vi "Stop Condition - Saturation 1 (SubVI) (1).vi"(6 "Enum":enum16{"Saturation", "B-Check"}(ring), 8 "error in (no error)":errorcluster, 9 "Test RunTime":dbl, 10 "Time":dbl, 11 "Cluster in":T1 {"M Event" items=["Stop", "Running", "PID", "Up Limit", "Down Limit", "Load Limit"]; "Test Type" items=["Please Select", "Triaxial Shear", "Triaxial UU", "Shearbox", "Permeability", "Consolidation (Stepped Loading)/Swelling", "Saturation (Incremental)", "User Defined", "UCT", "Isotropic Consolidation", "Swelling Pressure", "B-Check", "Saturation (Step Increment)", "Saturation (Ramp)"]; "Data"."Test Type" items=["Please Select", "Triaxial Shear", "Triaxial UU", "Shearbox", "Permeability", "Consolidation (Stepped Loading)/Swelling", "Saturation (Incremental)", "User Defined", "UCT", "Isotropic Consolidation", "Swelling Pressure", "B-Check", "Saturation (Step Increment)", "Saturation (Ramp)"]}) -> (0 "error out":errorcluster, 3 "Cluster out":T1 {"M Event" items=["Stop", "Running", "PID", "Up Limit", "Down Limit", "Load Limit"]; "Test Type" items=["Please Select", "Triaxial Shear", "Triaxial UU", "Shearbox", "Permeability", "Consolidation (Stepped Loading)/Swelling", "Saturation (Incremental)", "User Defined", "UCT", "Isotropic Consolidation", "Swelling Pressure", "B-Check", "Saturation (Step Increment)", "Saturation (Ramp)"]; "Data"."Test Type" items=["Please Select", "Triaxial Shear", "Triaxial UU", "Shearbox", "Permeability", "Consolidation (Stepped Loading)/Swelling", "Saturation (Incremental)", "User Defined", "UCT", "Isotropic Consolidation", "Swelling Pressure", "B-Check", "Saturation (Step Increment)", "Saturation (Ramp)"]}, 4 "Delay":string, 7 "Log?":bool)   [LabVIEW 2019]
uses:
  Controls/RunTest - Data Structure.ctl
  Controls/Test Panel - Data Structure.ctl
  Controls/Station - Test Type.ctl
  <vilib>/Utility/miscctls.llb/LVRowAndColumnTypeDef.ctl
  Controls/RunTest - Calculate Data.ctl
  <vilib>/httpClient/ClientHandle.ctl
  Controls/RunTest - Start Condition.ctl
  Controls/RunTest - Stop Condition.ctl
  Controls/UDP - Event.ctl
  Controls/eFGV States.ctl
  <vilib>/httpClient/LabVIEWHTTPClient.lvlib
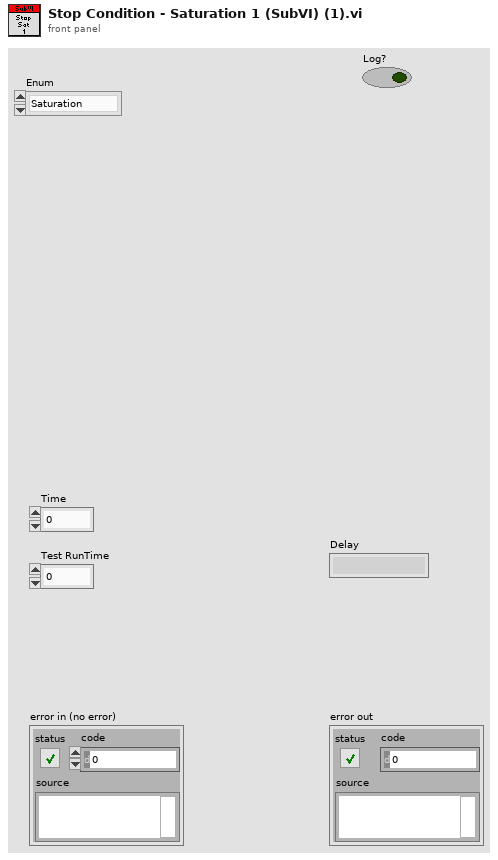
[diagram p1: front panel]
types:
  T1 = typedef "RunTest - Data Structure.ctl" = cluster{"Test Plan":string[], "PlanRow":i32, "Device Name":string[], "Timeout":i32, "Start?":bool, "Pause?":bool, "IP Address":string[], "LogRow":i32, "Logtype":u16, "Log Elapse":sgl, "Data":T2, "Stop log?":bool, "tdms":refnum<k34>, "Sensor Data":sgl[], "Start time":timestamp, "Prev Log Elapse":u32, "Plot":u16, "X-Axis":u16[], "Y-Axis":u16[], "XY":cluster{"X":dbl, "Y":dbl}[][], "End Stage?":bool, "1run":bool, "Condition":u16[], "Start Con":bool, "Log Con":bool, "Stop Con":bool, "Start Elapse":dbl, "Start Load":dbl, "Motor":i32, "StartRow":i32, "number log":i32, "Dir":bool, "Start time test":timestamp, "Auto":bool, "Check return?":bool, "Inv":cluster{"M":i32[], "Bool":bool[]}, "tdms temp":refnum<k34>, "Zero?":bool, "Plot Timer":dbl, "1st Run":bool, "TDMS Path":path, "MaxLoad":dbl, "Log Timer":sgl[], "Test Type":T3, "Log Sensor":string[], "Save?":bool, "1st Log":bool, "Y-Axis 2":u16[], "On Y-Axis 2":bool, "Decimal":u8[], "Init":cluster{"PWP TS":sgl, "Load TS":sgl, "Volume TS":sgl, "Disp TS":sgl, "CP":sgl, "Vol In":sgl, "Vol Out":sgl, "Load UCT":sgl, "Disp UCT":sgl, "PWP Sat":sgl, "CP Sat":sgl, "Volume IsoCons":sgl, "PWP IsoCons":sgl, "PWP TUU":sgl, "Load TUU":sgl, "Volume TUU":sgl, "Disp TUU":sgl, "Load Cons":sgl, "Disp Cons":sgl, "Volume Sat":sgl, "Vertical Load SB":sgl, "Vertical Disp SB":sgl, "H Disp SB":sgl, "H Load SB":sgl, "PWP BC":sgl, "CP BC":sgl, "PWP Sat Step":sgl, "CP Sat Step":sgl, "Volume Sat Step":sgl, "PWP Sat Ramp":sgl, "CP Sat Ramp":sgl, "Volume Sat Ramp":sgl}, "Calc":T5, "Device Index":i32[], "Channel Index":i32[], "http ref":T6, "fileid":string, "Step Cons":cluster{"V Stress":sgl, "H Settlement":sgl}, "RunTest":bool, "Graph Last":i32, "Init?":bool, "Datalog":bool[], "Start":T7, "Stop":T8, "Running?":bool, "StartTime":dbl, "Log Prev Time":dbl, "KeyName":string[], "Test RunTime":dbl, "Log Prev Axial":dbl, "M Event":T9[], "Last Log":bool, "popup":bool, "PreStart UU":bool, "PreStart Sat":bool, "PreStart BC":bool, "PreStart Sat Step":bool, "PreStart Sat Ramp":bool, "Prev Sat IP":string}
  T2 = typedef "Test Panel - Data Structure.ctl" = cluster{"Station":string, "Sample ID":string, "Job No":string, "Job Description":string, "Filename":string, "Test Type":T3, "Speciment No":string, "Depth":string, "Height":string, "Diameter/Length":string, "Weight":string, "Test Parameter":string, "Station[]":string[], "Edit Pos":T4, "Edit Pos Prev":T4, "Area":string, "Path":string, "sample_id":string}
  T3 = typedef "Station - Test Type.ctl" = u16
  T4 = typedef "LVRowAndColumnTypeDef.ctl" = cluster{"Row":i32, "Column":i32}
  T5 = typedef "RunTest - Calculate Data.ctl" = cluster{"TS":cluster{"Change PWP":sgl, "Change Vol":sgl, "Axial Load":sgl, "CiL":sgl, "Deviator":sgl, "Axial Strain":sgl, "MaxDeviator":sgl, "SS":sgl, "CAS":sgl}, "TUU":cluster{"Change PWP":sgl, "Axial Load":sgl, "CiL":sgl, "Deviator":sgl, "Axial Strain":sgl, "MaxDeviator":sgl}, "Sat":cluster{"B Value":sgl, "PWP Diss":sgl, "CPP":sgl, "CV":sgl}, "Per":cluster{"Change Vol In":sgl, "Change Vol Out":sgl, "Mean Vol":sgl, "Gradient Pressure":sgl, "Outlet Flow":sgl, "Inlet Flow":sgl, "I X1":sgl, "I X2":sgl, "I Y1":sgl, "I Y2":sgl, "O X1":sgl, "O X2":sgl, "O Y1":sgl, "O Y2":sgl}, "Step Cons":cluster{"V Stress":sgl, "H Settlement":sgl, "Total H Settle":sgl, "Prev Total H":sgl}, "UCT":cluster{"ALC":sgl, "H Change":sgl, "Deviator":sgl, "Axial Strain":sgl, "V Stress":sgl, "MaxDeviator":sgl}, "ISO Cons":cluster{"CPP":sgl, "PWP Diss":sgl, "CV":sgl, "VS":sgl}, "SB":cluster{"Speci LenC":sgl, "Shear Strain":sgl, "H LC":sgl, "Normal Stress":sgl, "Shear Stress":sgl, "MaxShear":sgl}, "BC":cluster{"B Value":sgl, "PWP Diss":sgl, "CPP":sgl, "CV":sgl}, "Sat Step":cluster{"B Value":sgl, "PWP Diss":sgl, "CPP":sgl, "CV":sgl}, "Sat Ramp":cluster{"B Value":sgl, "PWP Diss":sgl, "CPP":sgl, "CV":sgl}, "Prev Log":string[]}
  T6 = typedef "LabVIEWHTTPClient.lvlib/ClientHandle.ctl" = refnum<k1>
  T7 = typedef "RunTest - Start Condition.ctl" = cluster{"Cons":cluster{"VS":dbl, "Delay":bool, "No Delay":dbl}, "Sat":cluster{"CP":dbl, "BP":dbl, "StartBP":bool, "Target CP":bool, "Target BP":bool}, "Iso":cluster{"Select":dbl, "BP":dbl, "IC2":dbl, "IC3":dbl, "IC4":dbl, ". IC6":bool, "IC6":dbl, "IC6-2":dbl, "Time Cond":dbl, "Last PWP":dbl, "Target CP":bool, "Target BP":bool, "NewCP":dbl, "NewBP":dbl, "Noti CP":bool, "Noti BP":bool, "Noti PWP":bool, "PrevSatBP":dbl}, "TS":cluster{"SS":dbl, "Engage":bool, "ES":dbl, "LC":dbl, "PreStart":bool, "Trig SS":bool, "Drain":dbl, "Select":u16, "Max SS .":bool, "MaxSS":dbl}, "TUU":cluster{"SS":dbl, "Engage":bool, "ES":dbl, "LC":dbl, "PreStart":bool, "Trig SS":bool, "CP":dbl, "Delay Value":dbl, "Delay":bool, "CP PID":bool}, "UCT":cluster{"SS":dbl, "Engage":bool, "ES":dbl, "LC":dbl, "PreStart":bool, "Trig SS":bool}, "Enable?":bool, "SB":cluster{"SS":dbl, "Engage":bool, "ES":dbl, "LC":dbl, "PreStart":bool, "Trig SS":bool, "VS":dbl, "Delay Value":dbl, "Delay":bool, "VS PID":bool}, "Perm":cluster{"DP":dbl}, "BC":cluster{"CP":dbl, "Target CP":bool, "Target BP":bool, "CP Inc":dbl, "CP .Init":bool, "CP Init":dbl, "1st BC":bool}, "Sat (Step)":cluster{"Select":dbl, "CP":dbl, "BP":dbl, "EP":dbl, "StartCP":bool, "Target CP":bool, "Target BP":bool}, "Sat (Ramp)":cluster{"Select":dbl, "CP":dbl, "BP":dbl, "EP":dbl, "StartCP":bool, "Target CP":bool, "Target BP":bool, "Time Rate":u32}}
  T8 = typedef "RunTest - Stop Condition.ctl" = cluster{"Cons":cluster{"Select":i32, "Disp":dbl, "Time":dbl, "Time2":dbl, "Disp 2":dbl, "Time Cond":dbl, "Last Disp":dbl, "Swell":bool, "T50,90,100":cluster{"t50_x_min":dbl, "t50_y_value":dbl, "t90_x_min":dbl, "t90_y_value":dbl, "t100_x_min":dbl, "t100_y_value":dbl, "target_column":string, "test_type":string, "error":string}}, "Sat":cluster{"Select":i32, "PP":dbl, "Time":dbl, "VC":dbl, "Time2":dbl, "Time Cond":dbl, "Last PP":dbl, ".B":bool, "B":dbl, "Last Vc":dbl, "Time Cond 2":dbl, "Time3":dbl, "Time Cond 3":dbl, "B Achieve":bool, "PP Achieve":bool, "VC Achieve":bool, "Max Achieve":bool, "CP Check":dbl, "Skip Next":bool, "B Achieve Stage":u32, ".CP Check":bool}, "Iso":cluster{"PP":dbl, "Time":dbl, "VC":dbl, "Time2":dbl, "Time Cond":dbl, "Last Vc":dbl, ".PP":bool, "Time Cond 2":dbl, "Select":i32, "BS":cluster{"t50_x_min":dbl, "t50_y_value":dbl, "t90_x_min":dbl, "t90_y_value":dbl, "t100_x_min":dbl, "t100_y_value":dbl, "target_column":string, "test_type":string, "error":string}, "Final VC":dbl, "ASTM":cluster{"t50_x_min":dbl, "t50_y_value":dbl, "t90_x_min":dbl, "t90_y_value":dbl, "t100_x_min":dbl, "t100_y_value":dbl, "target_column":string, "test_type":string, "error":string}, "ASTM Log":cluster{"t50_x_min":dbl, "t50_y_value":dbl, "t90_x_min":dbl, "t90_y_value":dbl, "t100_x_min":dbl, "t100_y_value":dbl, "target_column":string, "test_type":string, "error":string}, "PP Achieve":bool, "VC Achieve":bool}, "TS":cluster{"Axial":dbl, ".MaxDev":bool, "MaxDev Value":dbl, "Return":bool, "Reset":bool, "Prev Time":dbl, "PostStop Run":bool, "CP Stop":bool, "BP Stop":bool, "PostStop Trig":bool, "Reset Value":dbl, "BPTrig":bool, "CPTrig":bool, "VLCTrig":bool, "CAxial":dbl, "Select":i32}, "TUU":cluster{"Axial":dbl, ".MaxDev":bool, "MaxDev Value":dbl, "Return":bool, "Reset":bool, "Prev Time":dbl, "PostStop Run":bool, "CP Stop":bool, "BP Stop":bool, "PostStop Trig":bool, "Reset Value":dbl, "BPTrig":bool, "CPTrig":bool, "VLCTrig":bool}, "UCT":cluster{"Axial":dbl, ".MaxDev":bool, "MaxDev Value":dbl, "Return":bool, "Reset":bool, "Prev Time":dbl, "PostStop Run":bool, "CP Stop":bool, "BP Stop":bool, "PostStop Trig":bool}, "Enable?":bool, "SB":cluster{"Shear":dbl, ".MaxShear":bool, "MaxShear Value":dbl, "Return":bool, "Reset":bool, "Prev Time":dbl, "PostStop Run":bool, "CP Stop":bool, "BP Stop":bool, "PostStop Trig":bool, "Reset Value":dbl, "BPTrig":bool, "CPTrig":bool, "VLCTrig":bool}, "Perm":cluster{"Max Time":bool, "Reset":bool, "PostStop Run":bool, "Ratio":bool, "Reset Value":dbl, "Time":dbl, "RatioTime":dbl, "RatioMore":dbl, "RatioLess":dbl, "Time Cond":dbl, "Time Cond 2":dbl, "Prev IF":dbl, "Prev OF":dbl, "PostStop Trig":bool, "BP Trig":bool, "DP Stop":bool, "BP Stop":bool, "CP Stop":bool, "CP Trig":bool}, "SP":cluster{".Max Time":bool, ".Time":bool, "Time":dbl, "MaxTime":dbl, "Time Cond":dbl, "Max Time Cond":dbl, "Stress":dbl}, "BC":cluster{"Select":i32, "PP":dbl, "Time":dbl, "Time Cond":dbl, "Last PP":dbl, ".B":bool, "B":dbl, "Time 2":dbl, "Time Cond 2":dbl, "B Achieve":bool, "PP Achieve":bool, "Max Achieve":bool, "CP Check":dbl, "Skip Next":bool, "B Achieve Stage":u32, ".CP Check":bool}, "Sat (Step)":cluster{"Select":i32, "PP":dbl, "Time":dbl, "VC":dbl, "Time2":dbl, "Time Cond":dbl, "Last PP":dbl, ".B":bool, "B":dbl, "Last Vc":dbl, "Time Cond 2":dbl, "Time3":dbl, "Time Cond 3":dbl, "B Achieve":bool, "PP Achieve":bool, "VC Achieve":bool, "Max Achieve":bool, "CP Check":dbl, "Skip Next":bool, "B Achieve Stage":u32}, "Sat (Ramp)":cluster{"Select":i32, "PP":dbl, "Time":dbl, "VC":dbl, "Time2":dbl, "Time Cond":dbl, "Last PP":dbl, ".B":bool, "B":dbl, "Last Vc":dbl, "Time Cond 2":dbl, "Time3":dbl, "Time Cond 3":dbl, "B Achieve":bool, "PP Achieve":bool, "VC Achieve":bool, "Max Achieve":bool, "CP Check":dbl, "Skip Next":bool, "B Achieve Stage":u32}}
  T9 = typedef "UDP - Event.ctl" = u16
  T10 = typedef "eFGV States.ctl" = enum16{"Init", "Read", "Write", "Exit"}
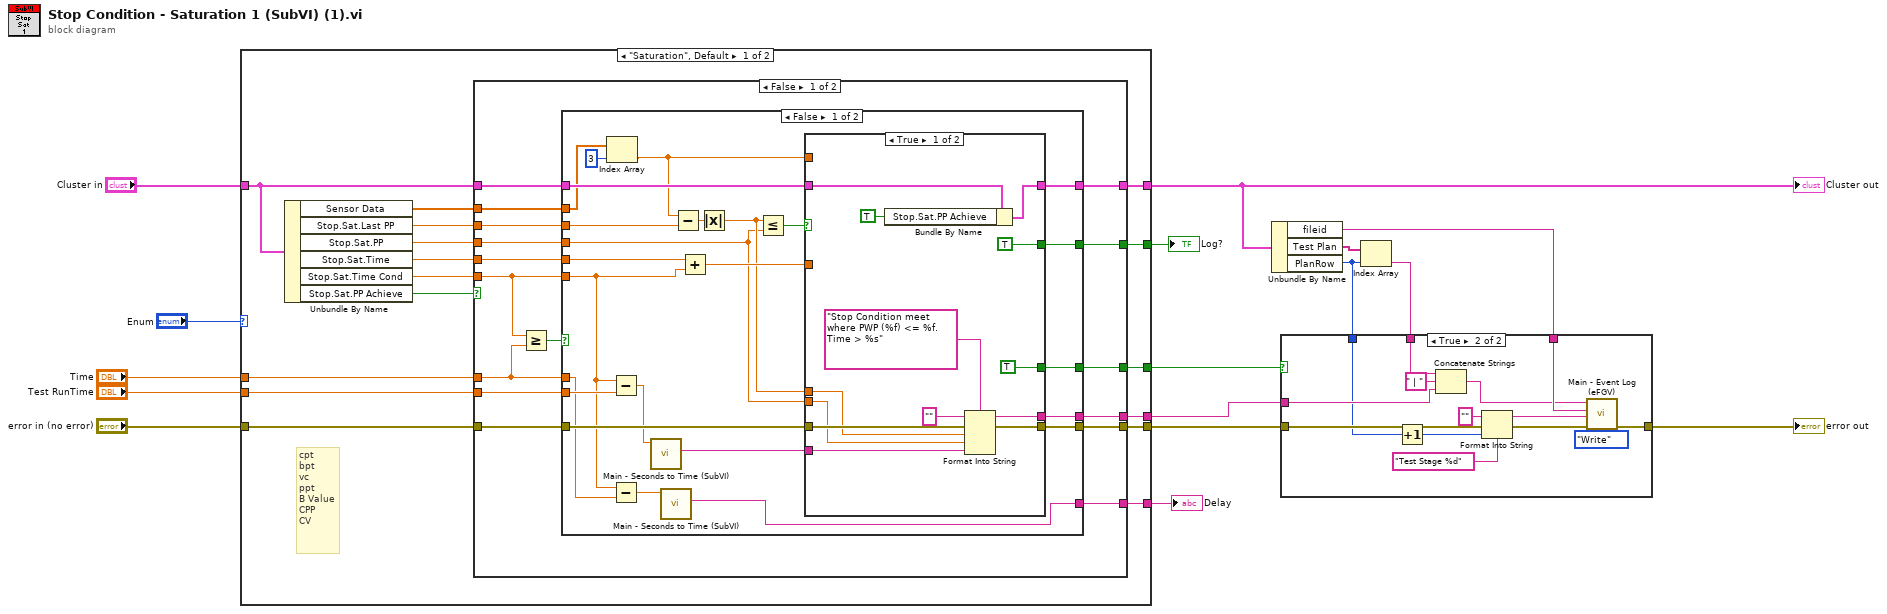
[diagram p0: block diagram]
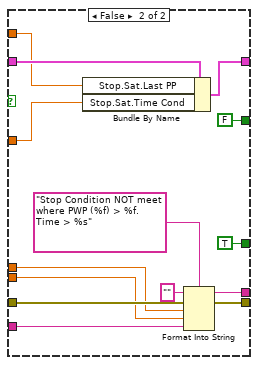
[diagram p2: hidden frame]
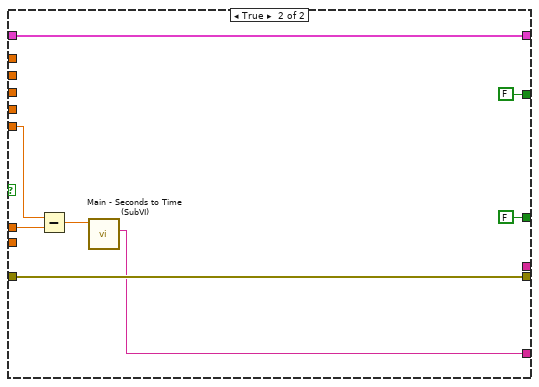
[diagram p3: hidden frame]
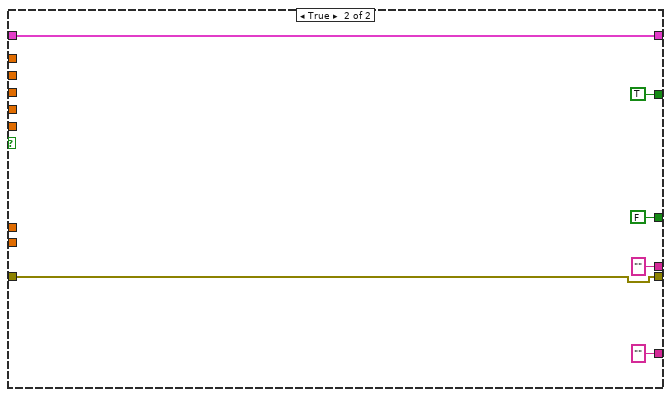
[diagram p4: hidden frame]
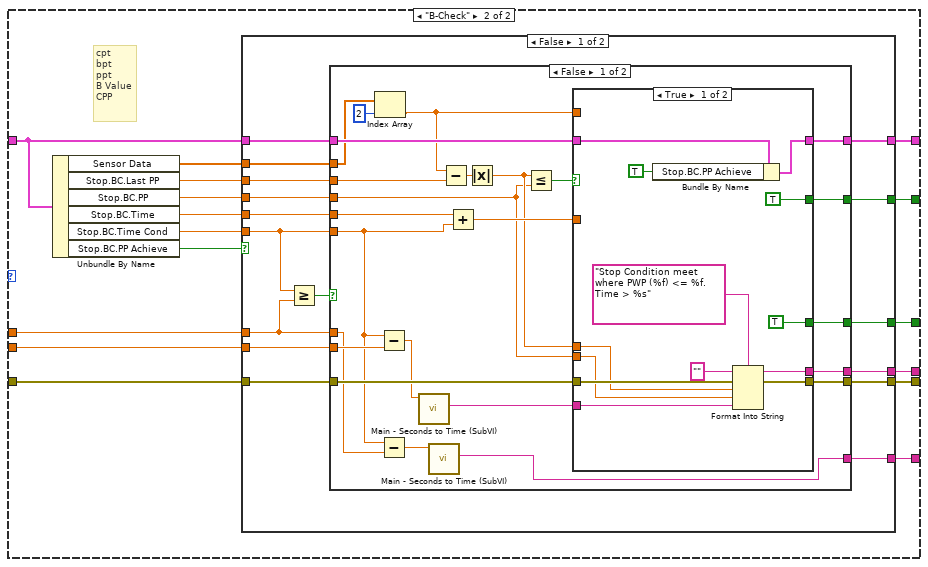
[diagram p5: hidden frame]
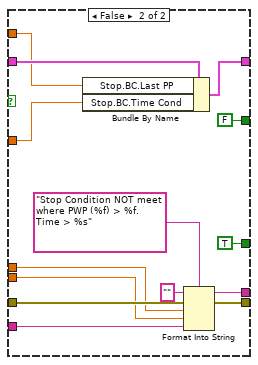
[diagram p6: hidden frame]
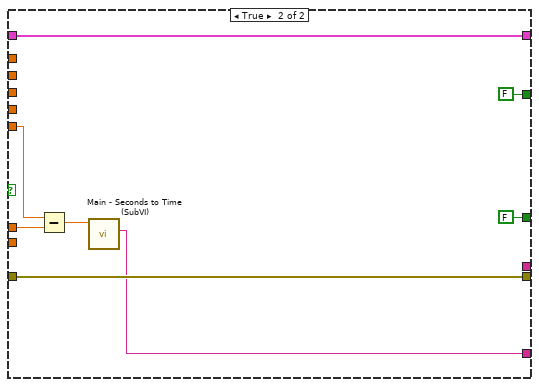
[diagram p7: hidden frame]
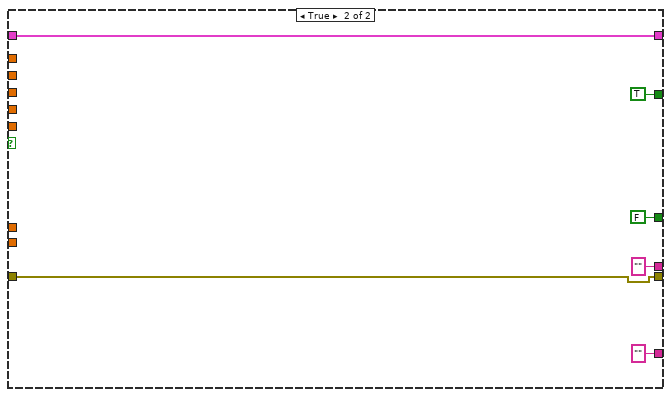
[diagram p8: hidden frame]
diagram:
  n1 = case shown="\"Saturation\", Default" "Enum" {
    tunnel: [w32 w129] -> w16
    tunnel: "Cluster in" -> [w26 w123]
    tunnel: "Test RunTime" -> [w25 w122]
    tunnel: "Time" -> [w24 w121]
    tunnel: "error in (no error)" -> [w23 w120]
    tunnel: [w22 w119] -> w11
    tunnel: [w20 w117] -> w6
    tunnel: [w19 w116] -> w5
    tunnel: [w18 w115] -> w4
    tunnel: [w17 w114] -> w3
    frame "Saturation", Default {
      # "cpt\nbpt\nvc\nppt\nB Value\nCPP\nCV"
      n2 = Unbundle By Name(w26) -> ("Sensor Data"=w27:sgl[], "Stop.Sat.Last PP"=w28:dbl, "Stop.Sat.PP"=w29:dbl, "Stop.Sat.Time"=w30:dbl, "Stop.Sat.Time Cond"=w31:dbl, "Stop.Sat.PP Achieve"=w21:bool)
      n3 = case shown="False" w21 {
        tunnel: [w48 "" ("Time string")] -> w32
        tunnel: w31 -> [w47 _]
        tunnel: w30 -> [w46 _]
        tunnel: w29 -> [w45 _]
        tunnel: w28 -> [w44 _]
        tunnel: w27 -> [w43 _]
        tunnel: w26 -> [w42 w113]
        tunnel: w25 -> [w41 _]
        tunnel: w24 -> [w40 _]
        tunnel: [w39 FALSE] -> w18
        tunnel: [w38 ""] -> w19
        tunnel: w23 -> [w37 w109]
        tunnel: [w35 w113] -> w17
        tunnel: [w34 w109] -> w20
        tunnel: [w33 TRUE] -> w22
        frame False {
          n4 = Greater Or Equal?(x=w47, y=w40) -> (x >= y?=w36:bool)
          n5 = case shown="False" w36 {
            tunnel: [w62 w107] -> w34
            tunnel: w37 -> [w63 w107]
            tunnel: [w72 w106] -> w35
            tunnel: w42 -> [w71 w106]
            tunnel: w44 -> [w69 _]
            tunnel: w45 -> [w58 _]
            tunnel: w46 -> [w57 _]
            tunnel: w47 -> [w53 w103]
            tunnel: w43 -> [w66 _]
            tunnel: [w61 _] -> w38
            tunnel: [w60 FALSE] -> w39
            tunnel: w40 -> [w52 w102]
            tunnel: w41 -> [w56 _]
            tunnel: [w50 w101] -> w48
            tunnel: [w49 FALSE] -> w33
            frame False {
              n6 = Index Array(array=w66, index=3) -> (element=w65:sgl)
              n7 = Subtract(x=w53, y=w56) -> (x-y=w55:dbl)
              n8 = Subtract(x=w53, y=w52) -> (x-y=w54:dbl)
              n9 = call "Main - Seconds to Time (SubVI).vi"("Seconds"=w55) -> ("Time string"=w51:string)  [unwired: 9 in, 1 out]
              n10 = call "Main - Seconds to Time (SubVI).vi"("Seconds"=w54) -> ("Time string"=w50:string)  [unwired: 9 in, 1 out]
              n11 = Subtract(x=w65, y=w69) -> (x-y=w68:dbl)
              n12 = Add(x=w57, y=w53) -> (x+y=w70:dbl)
              n13 = Absolute Value(x=w68) -> (abs(x)=w59:dbl)
              n14 = Less Or Equal?(x=w59, y=w58) -> (x <= y?=w67:bool)
              n15 = case shown="True" w67 {
                tunnel: [w75 w99] -> w72
                tunnel: w71 -> [w74 w98]
                tunnel: w70 -> [_ w97]
                tunnel: w65 -> [_ w96]
                tunnel: w63 -> [w84 w93]
                tunnel: [w83 w94] -> w62
                tunnel: [w82 w92] -> w61
                tunnel: [TRUE TRUE] -> w60
                tunnel: w59 -> [w80 w90]
                tunnel: w58 -> [w79 w89]
                tunnel: w51 -> [w78 w88]
                tunnel: [TRUE FALSE] -> w49
                frame True {
                  n16 = Bundle By Name(cluster=w74, "Stop.Sat.PP Achieve"=TRUE) -> (w75:T1)
                  n17 = Format Into String(format string="Stop Condition meet where PWP (%f) <= %f.  Time > %s", initial string="", error in=w84, w80, w79, w78) -> (resulting string=w82:string, error out=w83:errorcluster)
                }
                frame False {
                  n18 = Bundle By Name(cluster=w98, "Stop.Sat.Last PP"=w96, "Stop.Sat.Time Cond"=w97) -> (w99:T1)
                  n19 = Format Into String(format string="Stop Condition NOT meet where PWP (%f) > %f. Time > %s", initial string="", error in=w93, w90, w89, w88) -> (resulting string=w92:string, error out=w94:errorcluster)
                }
              }
            }
            frame True {
              n20 = Subtract(x=w103, y=w102) -> (x-y=w104:dbl)
              n21 = call "Main - Seconds to Time (SubVI).vi"("Seconds"=w104) -> ("Time string"=w101:string)  [unwired: 9 in, 1 out]
            }
          }
        }
        frame True {
        }
      }
    }
    frame "B-Check" {
      # "cpt\nbpt\nppt\nB Value\nCPP"
      n22 = Unbundle By Name(w123) -> ("Sensor Data"=w124:sgl[], "Stop.BC.Last PP"=w125:dbl, "Stop.BC.PP"=w126:dbl, "Stop.BC.Time"=w127:dbl, "Stop.BC.Time Cond"=w128:dbl, "Stop.BC.PP Achieve"=w118:bool)
      n23 = case shown="False" w118 {
        tunnel: [w145 "" ("Time string")] -> w129
        tunnel: w128 -> [w144 _]
        tunnel: w127 -> [w143 _]
        tunnel: w126 -> [w142 _]
        tunnel: w125 -> [w141 _]
        tunnel: w124 -> [w140 _]
        tunnel: w123 -> [w139 w210]
        tunnel: w122 -> [w138 _]
        tunnel: w121 -> [w137 _]
        tunnel: [w136 FALSE] -> w115
        tunnel: [w135 ""] -> w116
        tunnel: w120 -> [w134 w206]
        tunnel: [w132 w210] -> w114
        tunnel: [w131 w206] -> w117
        tunnel: [w130 TRUE] -> w119
        frame False {
          n24 = Greater Or Equal?(x=w144, y=w137) -> (x >= y?=w133:bool)
          n25 = case shown="False" w133 {
            tunnel: [w159 w204] -> w131
            tunnel: w134 -> [w160 w204]
            tunnel: [w169 w203] -> w132
            tunnel: w139 -> [w168 w203]
            tunnel: w141 -> [w166 _]
            tunnel: w142 -> [w155 _]
            tunnel: w143 -> [w154 _]
            tunnel: w144 -> [w150 w200]
            tunnel: w140 -> [w163 _]
            tunnel: [w158 _] -> w135
            tunnel: [w157 FALSE] -> w136
            tunnel: w137 -> [w149 w199]
            tunnel: w138 -> [w153 _]
            tunnel: [w147 w198] -> w145
            tunnel: [w146 FALSE] -> w130
            frame False {
              n26 = Index Array(array=w163, index=2) -> (element=w162:sgl)
              n27 = Subtract(x=w150, y=w153) -> (x-y=w152:dbl)
              n28 = Subtract(x=w150, y=w149) -> (x-y=w151:dbl)
              n29 = call "Main - Seconds to Time (SubVI).vi"("Seconds"=w152) -> ("Time string"=w148:string)  [unwired: 9 in, 1 out]
              n30 = call "Main - Seconds to Time (SubVI).vi"("Seconds"=w151) -> ("Time string"=w147:string)  [unwired: 9 in, 1 out]
              n31 = Subtract(x=w162, y=w166) -> (x-y=w165:dbl)
              n32 = Add(x=w154, y=w150) -> (x+y=w167:dbl)
              n33 = Absolute Value(x=w165) -> (abs(x)=w156:dbl)
              n34 = Less Or Equal?(x=w156, y=w155) -> (x <= y?=w164:bool)
              n35 = case shown="True" w164 {
                tunnel: [w172 w196] -> w169
                tunnel: w168 -> [w171 w195]
                tunnel: w167 -> [_ w194]
                tunnel: w162 -> [_ w193]
                tunnel: w160 -> [w181 w190]
                tunnel: [w180 w191] -> w159
                tunnel: [w179 w189] -> w158
                tunnel: [TRUE TRUE] -> w157
                tunnel: w156 -> [w177 w187]
                tunnel: w155 -> [w176 w186]
                tunnel: w148 -> [w175 w185]
                tunnel: [TRUE FALSE] -> w146
                frame True {
                  n36 = Bundle By Name(cluster=w171, "Stop.BC.PP Achieve"=TRUE ("Stop.Sat.PP Achieve")) -> (w172:T1)
                  n37 = Format Into String(format string="Stop Condition meet where PWP (%f) <= %f.  Time > %s", initial string="", error in=w181, w177, w176, w175) -> (resulting string=w179:string, error out=w180:errorcluster)
                }
                frame False {
                  n38 = Bundle By Name(cluster=w195, "Stop.BC.Last PP"=w193, "Stop.BC.Time Cond"=w194) -> (w196:T1)
                  n39 = Format Into String(format string="Stop Condition NOT meet where PWP (%f) > %f. Time > %s", initial string="", error in=w190, w187, w186, w185) -> (resulting string=w189:string, error out=w191:errorcluster)
                }
              }
            }
            frame True {
              n40 = Subtract(x=w200, y=w199) -> (x-y=w201:dbl)
              n41 = call "Main - Seconds to Time (SubVI).vi"("Seconds"=w201) -> ("Time string"=w198:string)  [unwired: 9 in, 1 out]
            }
          }
        }
        frame True {
        }
      }
    }
  }
  "Delay" <- w16
  "Cluster out" <- w3
  "Log?" <- w11
  n42 = Unbundle By Name(w3) -> ("fileid"=w8:string, "Test Plan"=w9:string[], "PlanRow"=w7:i32)
  n43 = Index Array(array=w9, index=w7) -> (element=w10:string)
  n44 = case shown="True" w4 {
    tunnel: w6 -> [w211 w215]
    tunnel: [w211 w224] -> w2
    tunnel: w8 -> [_ w223]
    tunnel: w5 -> [_ w219]
    tunnel: w10 -> [_ w222]
    tunnel: w7 -> [_ w213]
    frame False {
    }
    frame True {
      n45 = Increment(x=w213) -> (x+1=w217:i32)
      n46 = Concatenate Strings(w222, " | " ("string"), w219) -> (w220:string)
      n47 = Format Into String(format string="Test Stage %d", initial string="", error in=w215, w217) -> (resulting string=w214:string, error out=w216:errorcluster)
      n48 = call "Main - Event Log (eFGV).vi"("Action"=eFGV_States."Write", "error in"=w216, "Stage"=w214, "Fileid"=w223, "Data In"=w220) -> ("error out"=w224:errorcluster)  [unwired: 3 in, 3 out]
    }
  }
  "error out" <- w2
